vi "calPassY.vi"(8 "error in (no error)":errorcluster caption="错误输入（无错误）") -> ()   [LabVIEW 2025]
uses:
  global.vi
  System.Windows.Forms
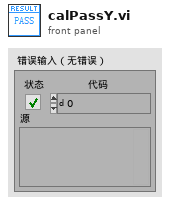
[diagram p1: front panel]
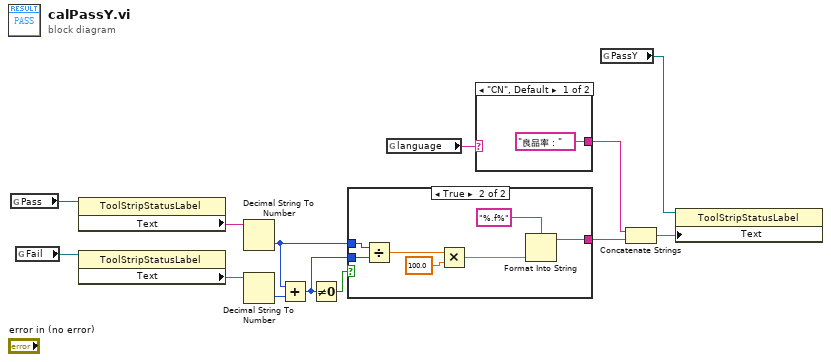
[diagram p0: block diagram]
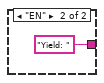
[diagram p2: hidden frame]
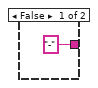
[diagram p3: hidden frame]
diagram:
  n1 = global read "global.vi" "Pass"() -> (w11:refnum<k24>)
  n2 = global read "global.vi" "Fail"() -> (w10:refnum<k24>)
  n3 = property class="ToolStripStatusLabel"(reference=w11) -> ("Text"=w9:string)  [unwired: 1 in, 2 out]
  n4 = property class="ToolStripStatusLabel"(reference=w10) -> ("Text"=w8:string)  [unwired: 1 in, 2 out]
  n5 = Decimal String To Number(string=w9) -> (number=w5:i32)  [unwired: 2 in, 1 out]
  n6 = Decimal String To Number(string=w8) -> (number=w7:i32)  [unwired: 2 in, 1 out]
  n7 = Add(x=w5, y=w7) -> (x+y=w6:i32)
  n8 = Not Equal To 0?(x=w6) -> (x != 0?=w12:bool)
  n9 = case shown="True" w12 {
    tunnel: ["-" w21] -> w2
    tunnel: w6 -> [_ w16]
    tunnel: w5 -> [_ w15]
    frame False {
    }
    frame True {
      n10 = Divide(x=w15, y=w16) -> (x/y=w19:dbl)
      n11 = Multiply(x=w19, y=100.0) -> (x*y=w18:dbl)
      n12 = Format Into String(format string="%.f%", w18) -> (resulting string=w21:string)  [unwired: 2 in, 1 out]
    }
  }
  n13 = global read "global.vi" "language"() -> (w4:string)
  n14 = case shown="\"CN\", Default" w4 {
    tunnel: ["良品率：" "Yield: "] -> w1
    frame "CN", Default {
    }
    frame "EN" {
    }
  }
  n15 = global read "global.vi" "PassY"() -> (w13:refnum<k24>)
  n16 = Concatenate Strings(w1, w2) -> (w3:string)
  n17 = property class="ToolStripStatusLabel"(reference=w13, "Text"=w3) -> ()  [unwired: 1 in, 2 out]
